vi "FinalProject.vi"() -> ()   [LabVIEW 2016]
uses:
  <vilib>/DAQmx/write.llb/DAQmx Write (Digital Bool 1Line 1Point).vi
  <vilib>/DAQmx/read.llb/DAQmx Read (Digital Bool 1Line 1Point).vi
  <vilib>/DAQmx/create/channels.llb/DAQmx Create Channel (DI-Digital Input).vi
  <vilib>/DAQmx/create/channels.llb/DAQmx Create Channel (DO-Digital Output).vi
  <vilib>/DAQmx/miscellaneous.llb/DAQmx Fill In Error Info.vi
panel:
  out "Pass Test":bool
  out "Overflow Status":bool
  out "Ring Count":i8
  in  "Write File":path
  out "Rejected Plastic":i32
  out "Rejected Metal":i32
  out "Odd Cases":i32
  out "Pass Product":i32
  out "Loading Status":bool
  out "Read File":string
  out "Write File":string
  out "Data Memory":string
  in  "Read File":path
  out "Ring Storage":i8(knob) scale=0.0..5.0
  in  "stop":bool
  out "Stop Button":bool
  out "Top Metal":bool
  out "Top Thing":bool
  out "Top Solenoid":bool
  out "Dropper Thing":bool
  out "Bottom Metal":bool
  out "Assembled":bool
  out "Bottom Solenoid":bool
  out "Bottom Thing":bool
  out "Start Button":bool
  in  "Reject Solenoid":bool
  in  "Belt motor":bool
  in  "Rotary":bool
  in  "Sort Solenoid":bool
  in  "Chain Motor":bool
  # "The overview structure of the program\n\n1. Start every with reading in from the file to retrieve the following data\n\n0: Number of rings in the holder\n1: Ring is loaded\n2: Number of rejeted plastic (Assembled: 0, Metal: 0)\n3: Number of rejected metal (Assembled: 0. Metal: 1)\n4: Number of odd case (Assembled: 1, Metal, 0)\n5: Number of passed product (Assembled: 1, Metal: 1)\n\n2. There are 3 major parts that run simutaneously together\n- Chain motors separates the plastic rings and metals. Exception is the number\nof rings is more than 5, there is nothing to push in (most needed data here)\n- Rotary to load the plastic ring when either there is at least one plastic ring and\nthe Dropper Thing detect empty\n- Assessment process\n\n3. Write in the same memory file in the same order when it started in tab\ndelimeter\n\n4. Repeat the cycle"
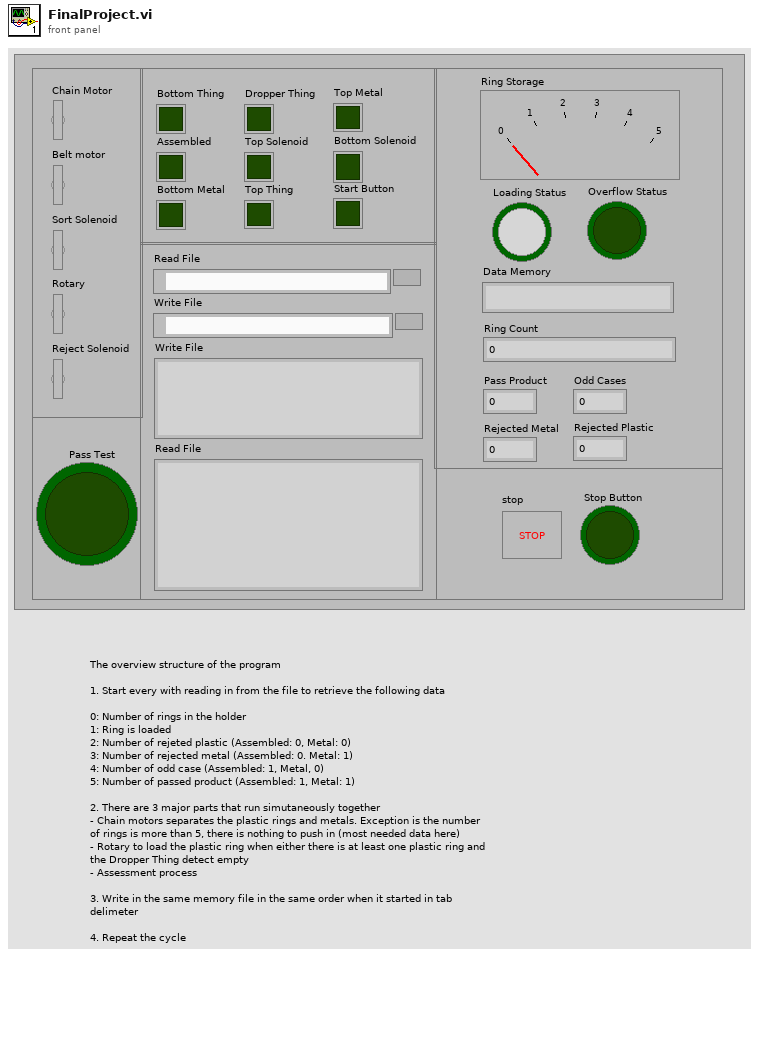
[diagram p1: front panel]
types:
  T1 = enum16{"open", "replace", "create", "open or create", "replace or create", "replace or create with confirmation"}
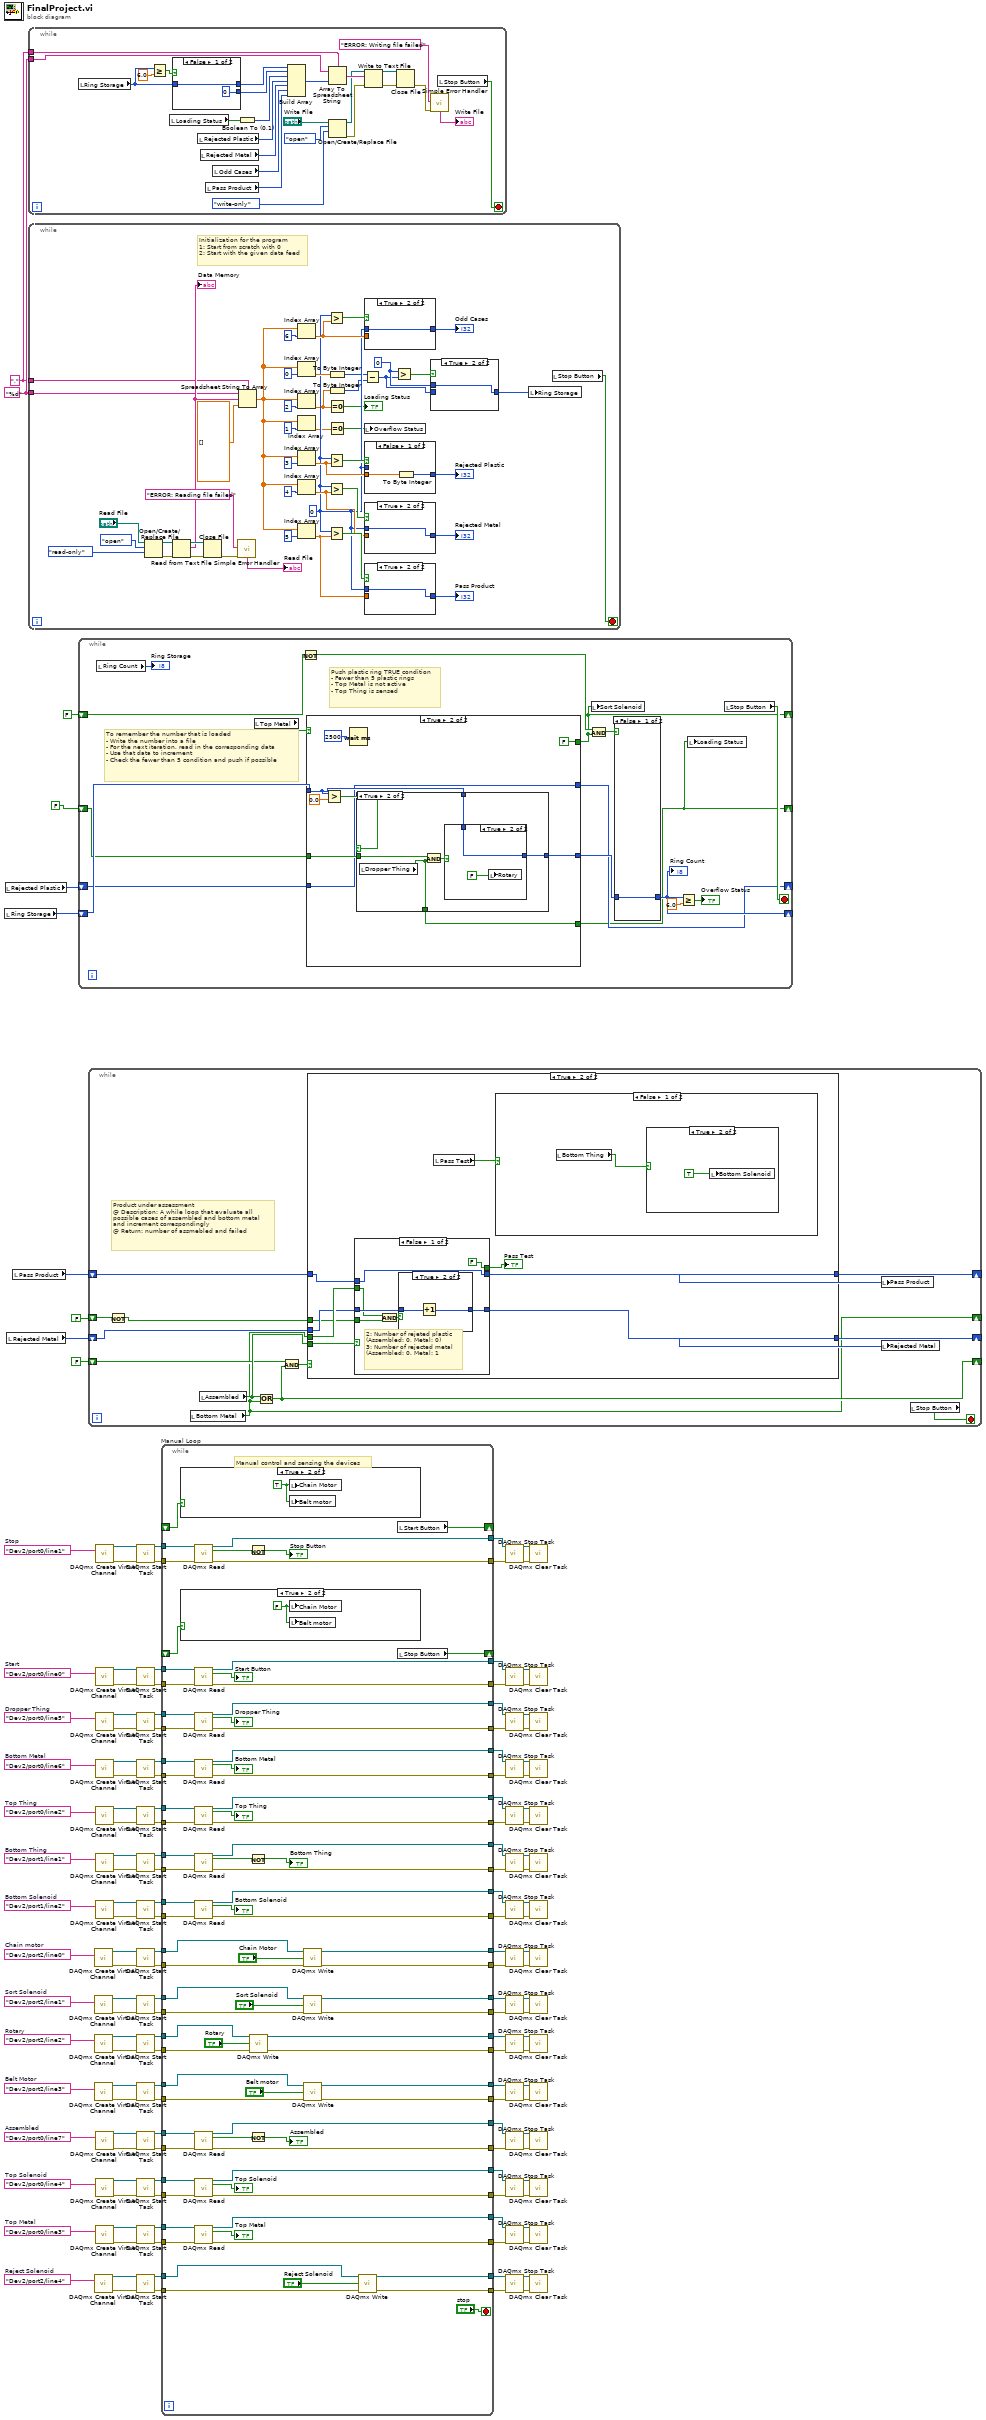
[diagram p0: block diagram]
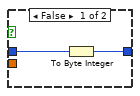
[diagram p2: hidden frame]
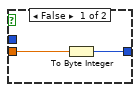
[diagram p3: hidden frame]
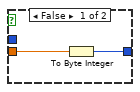
[diagram p4: hidden frame]
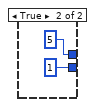
[diagram p7: hidden frame]
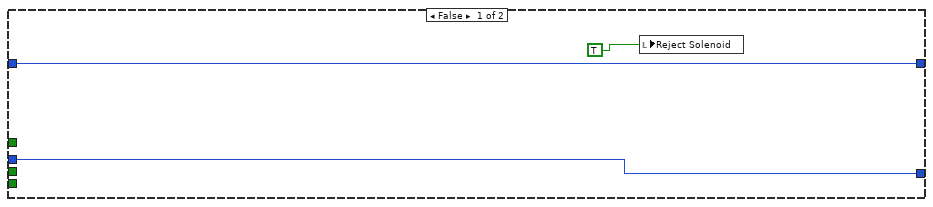
[diagram p8: hidden frame]
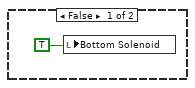
[diagram p9: hidden frame]
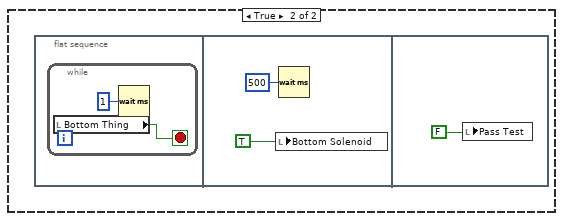
[diagram p10: hidden frame]
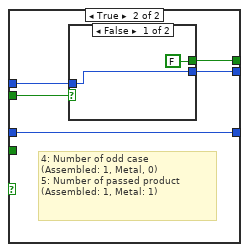
[diagram p12: hidden frame]
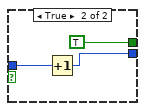
[diagram p13: hidden frame]
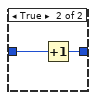
[diagram p14: hidden frame]
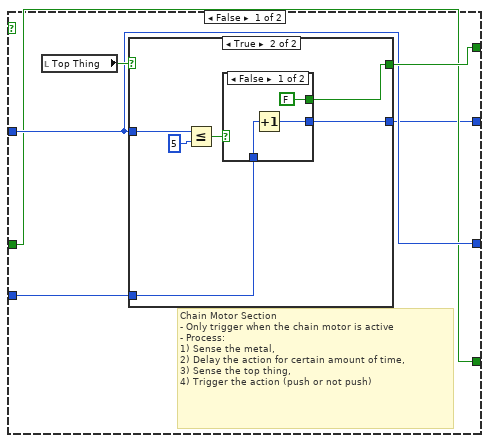
[diagram p15: hidden frame]
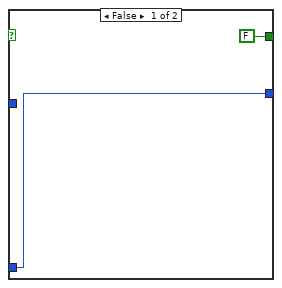
[diagram p16: hidden frame]
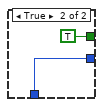
[diagram p17: hidden frame]
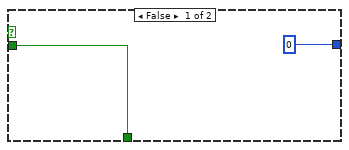
[diagram p18: hidden frame]
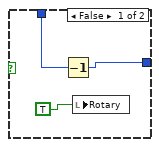
[diagram p19: hidden frame]
diagram:
  w9 = "," ("delimiter (Tab)")
  w10 = "%d" ("format string")
  w105 = tag "Dev2/port1/line2"  # Bottom Solenoid
  w106 = tag "Dev2/port1/line1"  # Bottom Thing
  w111 = tag "Dev2/port0/line7"  # Assembled
  w112 = tag "Dev2/port0/line6"  # Bottom Metal
  w117 = tag "Dev2/port0/line5"  # Dropper Thing
  w118 = tag "Dev2/port0/line4"  # Top Solenoid
  w123 = tag "Dev2/port0/line3"  # Top Metal
  w124 = tag "Dev2/port0/line2"  # Top Thing
  w127 = tag "Dev2/port2/line4"  # Reject Solenoid
  w132 = tag "Dev2/port2/line3"  # Belt Motor
  w133 = tag "Dev2/port2/line2"  # Rotary
  w142 = tag "Dev2/port2/line1"  # Sort Solenoid
  w143 = tag "Dev2/port2/line0"  # Chain motor
  w144 = tag "Dev2/port0/line1"  # Stop
  w145 = tag "Dev2/port0/line0"  # Start
  n1 = local read "Ring Storage"() -> (w8:i8)
  n2 = local read "Rejected Plastic"() -> (w2:i32)
  n3 = local read "Rejected Metal"() -> (w5:i32)
  n4 = local read "Pass Product"() -> (w4:i32)
  n5 = while {
    tunnel: w9 -> [w165]
    tunnel: w10 -> [w164]
    stop <- w157 stop-if-true
    n6 = local read "Ring Storage"() -> (w146:i8)
    n7 = Greater Or Equal?(x=w146, y=6.0) -> (x >= y?=w147:bool)
    n8 = local read "Loading Status"() -> (w155:bool)
    n9 = case shown="False" w147 {
      tunnel: [w172 5] -> w149
      tunnel: [0 1] -> w148
      tunnel: w146 -> [w172 _]
      frame False {
      }
      frame True {
      }
    }
    n10 = local read "Rejected Plastic"() -> (w154:i32)
    n11 = local read "Rejected Metal"() -> (w153:i32)
    n12 = local read "Pass Product"() -> (w151:i32)
    n13 = local read "Odd Cases"() -> (w152:i32)
    n14 = Boolean To (0,1)(Boolean=w155) -> (0, 1=w156:i16)
    n15 = Build Array(w149, w148, w156, w154, w153, w152, w151) -> (w163:i32[])
    n16 = Array To Spreadsheet String(delimiter (Tab)=w165, array=w163, 3:w164) -> (spreadsheet string=w166:string)
    n17 = Open/Create/Replace File(file path (use dialog)="Write File", operation (0:open)=T1."open", access (0:read/write)=enum16{"read/write", "read-only", "write-only"}."write-only") -> (refnum out=w159:refnum<file>, error out=w158:errorcluster)  [unwired: 3 in, 1 out]
    n18 = Write to Text File(file (use dialog)=w159, text=w166, error in=w158) -> (refnum out=w169:refnum<file>, error out=w168:errorcluster)  [unwired: 1 in, 1 out]
    n19 = Close File(refnum=w169, error in=w168) -> (error out=w171:errorcluster)  [unwired: 1 out]
    n20 = call <vilib>:"Simple Error Handler.vi"("error source (\" \")"="ERROR: Writing file failed", "error in (no error)"=w171) -> ("message"=→"Write File":string)  [unwired: 3 in, 4 out]
    n21 = local read "Stop Button"() -> (w157:bool)
  }
  n22 = while {
    tunnel: w10 -> [w192]
    tunnel: w9 -> [w191]
    stop <- w182 stop-if-true
    w205 = 0
    w218 = 0
    # "Initialization for the program\n1: Start from scratch with 0\n2: Start with the given data feed"
    n23 = Open/Create/Replace File(file path (use dialog)="Read File", operation (0:open)=T1."open", access (0:read/write)=enum16{"read/write", "read-only", "write-only"}."read-only") -> (refnum out=w204:refnum<file>, error out=w203:errorcluster)  [unwired: 3 in, 1 out]
    n24 = Read from Text File(file (use dialog)=w204, error in=w203) -> (refnum out=w198:refnum<file>, text=w193:string, error out=w202:errorcluster)  [unwired: 2 in, 1 out]
    "Data Memory" <- w193
    n25 = Close File(refnum=w198, error in=w202) -> (error out=w196:errorcluster)  [unwired: 1 out]
    n26 = call <vilib>:"Simple Error Handler.vi"("error source (\" \")"="ERROR: Reading file failed", "error in (no error)"=w196) -> ("message"=→"Read File":string)  [unwired: 3 in, 4 out]
    n27 = Spreadsheet String To Array(delimiter (Tab)=w191, format string=w192, spreadsheet string=w193, array type (2D Dbl)=dbl[] []) -> (array=w179:dbl[])
    n28 = Index Array(array=w179, index=6) -> (element=w206:dbl)
    n29 = Index Array(array=w179, index=0 ("index (vol)")) -> (element=w222:dbl)
    n30 = Index Array(array=w179, index=2) -> (element=w186:dbl)
    n31 = Index Array(array=w179, index=1 ("index (vol)")) -> (element=w176:dbl)
    n32 = Index Array(array=w179, index=3) -> (element=w209:dbl)
    n33 = Index Array(array=w179, index=4) -> (element=w208:dbl)
    n34 = Index Array(array=w179, index=5) -> (element=w207:dbl)
    n35 = Greater?(x=w205, y=w206) -> (0:w210:bool)
    n36 = Greater?(x=w205, y=w209) -> (0:w213:bool)
    n37 = Greater?(x=w205, y=w208) -> (0:w212:bool)
    n38 = Greater?(x=w205, y=w207) -> (0:w211:bool)
    n39 = To Byte Integer(number=w222) -> (8bit integer=w185:i8)
    n40 = To Byte Integer(number=w186) -> (8bit integer=w184:i8)
    n41 = Equal To 0?(x=w186) -> (x = 0?=→"Loading Status":bool)
    n42 = Equal To 0?(x=w176) -> (x = 0?=w177:bool)
    n43 = Subtract(x=w185, y=w184) -> (x-y=w183:i8)
    n44 = case shown="True" w210 {
      tunnel: [w224 w225] -> w187
      tunnel: w206 -> [_ _]
      tunnel: w205 -> [w223 w225]
      frame False {
        n45 = To Byte Integer(number=w223) -> (8bit integer=w224:i8)
      }
      frame True {
      }
    }
    "Odd Cases" <- w187
    n46 = local write "Overflow Status"(w177) -> ()
    n47 = case shown="False" w213 {
      tunnel: [w232 w234] -> w190
      tunnel: w205 -> [_ w234]
      tunnel: w209 -> [w233 _]
      frame False {
        n48 = To Byte Integer(number=w233) -> (8bit integer=w232:i8)
      }
      frame True {
      }
    }
    "Rejected Plastic" <- w190
    n49 = case shown="True" w212 {
      tunnel: [w229 w231] -> w189
      tunnel: w205 -> [_ w231]
      tunnel: w208 -> [w230 _]
      frame False {
        n50 = To Byte Integer(number=w230) -> (8bit integer=w229:i8)
      }
      frame True {
      }
    }
    "Rejected Metal" <- w189
    n51 = case shown="True" w211 {
      tunnel: [w226 w228] -> w188
      tunnel: w205 -> [_ w228]
      tunnel: w207 -> [w227 _]
      frame False {
        n52 = To Byte Integer(number=w227) -> (8bit integer=w226:i8)
      }
      frame True {
      }
    }
    "Pass Product" <- w188
    n53 = Greater?(x=w218, y=w183) -> (0:w219:bool)
    n54 = case shown="True" w219 {
      tunnel: [w235 w236] -> w181
      tunnel: w218 -> [_ w236]
      tunnel: w183 -> [w235 _]
      frame False {
      }
      frame True {
      }
    }
    n55 = local write "Ring Storage"(w181) -> ()
    n56 = local read "Stop Button"() -> (w182:bool)
  }
  n57 = while {
    shift-right: [w242] -> _
    shift-left: w8 -> [w250]
    shift-right: [w246] -> _
    shift-left: FALSE -> [w247]
    shift-right: [w237] -> _
    shift-left: FALSE -> [w241]
    shift-right: [w238] -> _
    shift-left: w2 -> [w239]
    stop <- w251 stop-if-true
    # "Push plastic ring TRUE condition\n- Fewer than 5 plastic rings\n- Top Metal is not active\n- Top Thing is sensed"
    # "To remember the number that is loaded\n- Write the number into a file\n- For the next iteration, read in the corresponding data\n- Use that data to increment\n- Check the fewer than 5 condition and push if possible"
    n58 = local read "Ring Count"() -> (→"Ring Storage":i8)
    n59 = local read "Top Metal"() -> (w252:bool)
    n60 = Not(x=w247) -> (.not. x?=w248:bool)
    n61 = case shown="True" w252 {
      tunnel: [w260 FALSE] -> w246
      tunnel: w250 -> [w259 w277]
      tunnel: w241 -> [w258 w279]
      tunnel: [w258 w278] -> w237
      tunnel: [w259 w276] -> w240
      tunnel: w239 -> [w257 w275]
      tunnel: [w256 w275] -> w238
      frame False {
        # "Chain Motor Section\n- Only trigger when the chain motor is active\n- Process: \n1) Sense the metal, \n2) Delay the action for certain amount of time, \n3) Sense the top thing,\n4) Trigger the action (push or not push)"
        n62 = local read "Top Thing"() -> (w261:bool)
        n63 = case shown="True" w261 {
          tunnel: [FALSE w267] -> w260
          tunnel: w259 -> [_ w266]
          tunnel: w257 -> [w262 w265]
          tunnel: [w262 w264] -> w256
          frame False {
          }
          frame True {
            n64 = Less Or Equal?(x=w266, y=i8 5) -> (x <= y?=w268:bool)
            n65 = case shown="False" w268 {
              tunnel: [FALSE TRUE] -> w267
              tunnel: w265 -> [w271 w273]
              tunnel: [w270 w273] -> w264
              frame False {
                n66 = Increment(x=w271) -> (x+1=w270:i32)
              }
              frame True {
              }
            }
          }
        }
      }
      frame True {
        n67 = Greater?(x=w277, y=0.0) -> (0:w280:bool)
        n68 = Wait (ms)(milliseconds to wait=u32 2500 ("millisecond timer value")) -> ()  [unwired: 1 out]
        n69 = case shown="True" w280 {
          tunnel: w279 -> [w284 w289]
          tunnel: [w284 w288] -> w278
          tunnel: w277 -> [_ w287]
          tunnel: [0 w286] -> w276
          frame False {
          }
          frame True {
            n70 = local read "Dropper Thing"() -> (w288:bool)
            n71 = And(x=w289, y=w288) -> (x .and. y?=w290:bool)
            n72 = case shown="True" w290 {
              tunnel: w287 -> [w292 w295]
              tunnel: [w293 w295] -> w286
              frame False {
                n73 = Decrement(x=w292) -> (x-1=w293:i32)
                n74 = local write "Rotary"(TRUE) -> ()
              }
              frame True {
                n75 = local write "Rotary"(FALSE) -> ()
              }
            }
          }
        }
      }
    }
    n76 = And(x=w248, y=w246) -> (x .and. y?=w249:bool)
    n77 = local write "Sort Solenoid"(w246) -> ()
    n78 = case shown="False" w249 {
      tunnel: [w253 w254] -> w242
      tunnel: w240 -> [w253 w255]
      frame False {
      }
      frame True {
        n79 = Increment(x=w255) -> (x+1=w254:i32)
      }
    }
    "Ring Count" <- w242
    n80 = Greater Or Equal?(x=w242, y=6.0) -> (x >= y?=→"Overflow Status":bool)
    n81 = local write "Loading Status"(w237) -> ()
    n82 = local read "Stop Button"() -> (w251:bool)
  }
  n83 = while {
    shift-right: [w303] -> _
    shift-left: FALSE -> [w305]
    shift-right: [w300] -> _
    shift-left: w5 -> [w302]
    shift-right: [w299] -> _
    shift-left: w4 -> [w301]
    shift-right: [w296] -> _
    shift-left: FALSE -> [w298]
    stop <- w307 stop-if-true
    # "Product under assessment\n@ Description: A while loop that evaluate all \npossible cases of assembled and bottom metal\nand increment correspondingly\n@ Return: number of assmebled and failed"
    n84 = Not(x=w298) -> (.not. x?=w297:bool)
    n85 = local read "Bottom Metal"() -> (w296:bool)
    n86 = local read "Assembled"() -> (w306:bool)
    n87 = Or(x=w306, y=w296) -> (x .or. y?=w303:bool)
    n88 = And(x=w305, y=w303) -> (x .and. y?=w304:bool)
    n89 = case shown="True" w304 {
      tunnel: w306 -> [_ w316]
      tunnel: w296 -> [_ w317]
      tunnel: w302 -> [w310 w315]
      tunnel: w301 -> [w309 w319]
      tunnel: [w310 w314] -> w300
      tunnel: [w309 w318] -> w299
      tunnel: w297 -> [_ w311]
      frame False {
        n90 = local write "Reject Solenoid"(TRUE) -> ()
      }
      frame True {
        n91 = case shown="False" w316 {
          tunnel: w319 -> [w334 w339]
          tunnel: [w334 w342] -> w318
          tunnel: w317 -> [w329 w341]
          tunnel: w315 -> [w333 w340]
          tunnel: [w332 w340] -> w314
          tunnel: [FALSE w338] -> w312
          tunnel: w311 -> [w328 _]
          frame False {
            # "2: Number of rejeted plastic\n(Assembled: 0, Metal: 0)\n3: Number of rejected metal\n(Assembled: 0. Metal: 1"
            n92 = And(x=w329, y=w328) -> (x .and. y?=w330:bool)
            n93 = case shown="True" w330 {
              tunnel: w333 -> [w335 w337]
              tunnel: [w335 w336] -> w332
              frame False {
              }
              frame True {
                n94 = Increment(x=w337) -> (x+1=w336:i32)
              }
            }
          }
          frame True {
            # "4: Number of odd case\n(Assembled: 1, Metal, 0)\n5: Number of passed product\n(Assembled: 1, Metal: 1)"
            n95 = case shown="False" w341 {
              tunnel: w339 -> [w344 w346]
              tunnel: [w344 w347] -> w342
              tunnel: [FALSE TRUE] -> w338
              frame False {
              }
              frame True {
                n96 = Increment(x=w346) -> (x+1=w347:i32)
              }
            }
          }
        }
        "Pass Test" <- w312
        n97 = local read "Pass Test"() -> (w313:bool)
        n98 = case shown="False" w313 {
          frame False {
            n99 = local read "Bottom Thing"() -> (w320:bool)
            n100 = case shown="True" w320 {
              frame False {
                n101 = local write "Bottom Solenoid"(TRUE) -> ()
              }
              frame True {
                n102 = local write "Bottom Solenoid"(TRUE) -> ()
              }
            }
          }
          frame True {
            n103 = flat-sequence {
              frame #0 {
                n104 = while {
                  stop <- w323 stop-if-true
                  n105 = local read "Bottom Thing"() -> (w323:bool)
                  n106 = Wait (ms)(milliseconds to wait=u32 1) -> ()  [unwired: 1 out]
                }
              }
              frame #1 {
                n107 = local write "Bottom Solenoid"(TRUE) -> ()
                n108 = Wait (ms)(milliseconds to wait=u32 500) -> ()  [unwired: 1 out]
              }
              frame #2 {
                n109 = local write "Pass Test"(FALSE) -> ()
              }
            }
          }
        }
      }
    }
    n110 = local write "Pass Product"(w299) -> ()
    n111 = local write "Rejected Metal"(w300) -> ()
    n112 = local read "Stop Button"() -> (w307:bool)
  }
  n113 = call-poly <vilib>:"DAQmx Create Virtual Channel.vi"("lines"=w143) -> ("task out"=w137:refnum<k21>, "error out"=w136:errorcluster)  [unwired: 13 in]
  n114 = call-poly <vilib>:"DAQmx Create Virtual Channel.vi"("lines"=w142) -> ("task out"=w135:refnum<k21>, "error out"=w134:errorcluster)  [unwired: 13 in]
  n115 = call-poly <vilib>:"DAQmx Create Virtual Channel.vi"("lines"=w133) -> ("task out"=w131:refnum<k21>, "error out"=w130:errorcluster)  [unwired: 13 in]
  n116 = call-poly <vilib>:"DAQmx Create Virtual Channel.vi"("lines"=w132) -> ("task out"=w129:refnum<k21>, "error out"=w128:errorcluster)  [unwired: 13 in]
  n117 = call-poly <vilib>:"DAQmx Create Virtual Channel.vi"("lines"=w127) -> ("task out"=w126:refnum<k21>, "error out"=w125:errorcluster)  [unwired: 13 in]
  n118 = call-poly <vilib>:"DAQmx Create Virtual Channel.vi"("lines"=w144) -> ("task out"=w139:refnum<k21>, "error out"=w138:errorcluster)  [unwired: 13 in]
  n119 = call-poly <vilib>:"DAQmx Create Virtual Channel.vi"("lines"=w145) -> ("task out"=w140:refnum<k21>, "error out"=w141:errorcluster)  [unwired: 13 in]
  n120 = call-poly <vilib>:"DAQmx Create Virtual Channel.vi"("lines"=w117) -> ("task out"=w114:refnum<k21>, "error out"=w113:errorcluster)  [unwired: 13 in]
  n121 = call-poly <vilib>:"DAQmx Create Virtual Channel.vi"("lines"=w112) -> ("task out"=w109:refnum<k21>, "error out"=w110:errorcluster)  [unwired: 13 in]
  n122 = call-poly <vilib>:"DAQmx Create Virtual Channel.vi"("lines"=w124) -> ("task out"=w121:refnum<k21>, "error out"=w122:errorcluster)  [unwired: 13 in]
  n123 = call-poly <vilib>:"DAQmx Create Virtual Channel.vi"("lines"=w106) -> ("task out"=w103:refnum<k21>, "error out"=w104:errorcluster)  [unwired: 13 in]
  n124 = call-poly <vilib>:"DAQmx Create Virtual Channel.vi"("lines"=w105) -> ("task out"=w102:refnum<k21>, "error out"=w101:errorcluster)  [unwired: 13 in]
  n125 = call-poly <vilib>:"DAQmx Create Virtual Channel.vi"("lines"=w111) -> ("task out"=w108:refnum<k21>, "error out"=w107:errorcluster)  [unwired: 13 in]
  n126 = call-poly <vilib>:"DAQmx Create Virtual Channel.vi"("lines"=w118) -> ("task out"=w115:refnum<k21>, "error out"=w116:errorcluster)  [unwired: 13 in]
  n127 = call-poly <vilib>:"DAQmx Create Virtual Channel.vi"("lines"=w123) -> ("task out"=w120:refnum<k21>, "error out"=w119:errorcluster)  [unwired: 13 in]
  n128 = call <vilib>:"DAQmx Start Task.vi"("task/channels in"=w139, "error in"=w138) -> ("task out"=w98:refnum<k21>, "error out"=w97:errorcluster)  [unwired: 12 in]
  n129 = call <vilib>:"DAQmx Start Task.vi"("task/channels in"=w140, "error in"=w141) -> ("task out"=w100:refnum<k21>, "error out"=w99:errorcluster)  [unwired: 12 in]
  n130 = call <vilib>:"DAQmx Start Task.vi"("task/channels in"=w114, "error in"=w113) -> ("task out"=w37:refnum<k21>, "error out"=w38:errorcluster)  [unwired: 12 in]
  n131 = call <vilib>:"DAQmx Start Task.vi"("task/channels in"=w109, "error in"=w110) -> ("task out"=w40:refnum<k21>, "error out"=w39:errorcluster)  [unwired: 12 in]
  n132 = call <vilib>:"DAQmx Start Task.vi"("task/channels in"=w121, "error in"=w122) -> ("task out"=w88:refnum<k21>, "error out"=w87:errorcluster)  [unwired: 12 in]
  n133 = call <vilib>:"DAQmx Start Task.vi"("task/channels in"=w103, "error in"=w104) -> ("task out"=w54:refnum<k21>, "error out"=w53:errorcluster)  [unwired: 12 in]
  n134 = call <vilib>:"DAQmx Start Task.vi"("task/channels in"=w102, "error in"=w101) -> ("task out"=w50:refnum<k21>, "error out"=w49:errorcluster)  [unwired: 12 in]
  n135 = call <vilib>:"DAQmx Start Task.vi"("task/channels in"=w137, "error in"=w136) -> ("task out"=w30:refnum<k21>, "error out"=w29:errorcluster)  [unwired: 12 in]
  n136 = call <vilib>:"DAQmx Start Task.vi"("task/channels in"=w135, "error in"=w134) -> ("task out"=w28:refnum<k21>, "error out"=w27:errorcluster)  [unwired: 12 in]
  n137 = call <vilib>:"DAQmx Start Task.vi"("task/channels in"=w131, "error in"=w130) -> ("task out"=w12:refnum<k21>, "error out"=w11:errorcluster)  [unwired: 12 in]
  n138 = call <vilib>:"DAQmx Start Task.vi"("task/channels in"=w129, "error in"=w128) -> ("task out"=w16:refnum<k21>, "error out"=w15:errorcluster)  [unwired: 12 in]
  n139 = call <vilib>:"DAQmx Start Task.vi"("task/channels in"=w108, "error in"=w107) -> ("task out"=w46:refnum<k21>, "error out"=w45:errorcluster)  [unwired: 12 in]
  n140 = call <vilib>:"DAQmx Start Task.vi"("task/channels in"=w115, "error in"=w116) -> ("task out"=w34:refnum<k21>, "error out"=w33:errorcluster)  [unwired: 12 in]
  n141 = call <vilib>:"DAQmx Start Task.vi"("task/channels in"=w120, "error in"=w119) -> ("task out"=w80:refnum<k21>, "error out"=w79:errorcluster)  [unwired: 12 in]
  n142 = call <vilib>:"DAQmx Start Task.vi"("task/channels in"=w126, "error in"=w125) -> ("task out"=w22:refnum<k21>, "error out"=w21:errorcluster)  [unwired: 12 in]
  n143 = while "Manual Loop" {
    tunnel: w100 -> [w429]
    tunnel: w99 -> [w428]
    tunnel: w98 -> [w425]
    tunnel: w97 -> [w424]
    tunnel: [w423] -> w94
    tunnel: [w422] -> w93
    tunnel: [w421] -> w90
    tunnel: [w420] -> w89
    tunnel: w88 -> [w419]
    tunnel: w87 -> [w418]
    tunnel: [w417] -> w84
    tunnel: [w416] -> w83
    tunnel: w80 -> [w415]
    tunnel: w79 -> [w414]
    tunnel: [w413] -> w78
    tunnel: [w412] -> w77
    tunnel: w54 -> [w411]
    tunnel: w53 -> [w410]
    tunnel: [w409] -> w52
    tunnel: [w408] -> w51
    tunnel: w50 -> [w407]
    tunnel: w49 -> [w406]
    tunnel: [w405] -> w48
    tunnel: [w404] -> w47
    tunnel: w46 -> [w402]
    tunnel: w45 -> [w401]
    tunnel: [w400] -> w44
    tunnel: [w399] -> w43
    tunnel: [w398] -> w42
    tunnel: [w397] -> w41
    tunnel: w40 -> [w396]
    tunnel: w39 -> [w395]
    tunnel: w38 -> [w394]
    tunnel: w37 -> [w393]
    tunnel: [w392] -> w36
    tunnel: [w391] -> w35
    tunnel: w34 -> [w390]
    tunnel: w33 -> [w389]
    tunnel: [w388] -> w32
    tunnel: [w387] -> w31
    tunnel: w30 -> [w386]
    tunnel: w29 -> [w385]
    tunnel: w28 -> [w384]
    tunnel: w27 -> [w383]
    tunnel: [w382] -> w26
    tunnel: [w381] -> w25
    tunnel: [w380] -> w24
    tunnel: [w379] -> w23
    tunnel: w22 -> [w378]
    tunnel: w21 -> [w377]
    tunnel: [w376] -> w20
    tunnel: [w375] -> w19
    tunnel: [w374] -> w18
    tunnel: [w373] -> w17
    tunnel: w16 -> [w372]
    tunnel: w15 -> [w371]
    tunnel: [w370] -> w14
    tunnel: [w369] -> w13
    tunnel: w12 -> [w368]
    tunnel: w11 -> [w367]
    shift-right: [w362] -> _
    shift-left: _ -> [w357]
    shift-right: [w361] -> _
    shift-left: _ -> [w358]
    stop <- "stop" stop-if-true
    # "Manual control and sensing the devices"
    n144 = case shown="True" w357 {
      frame False {
      }
      frame True {
        w431 = TRUE
        n145 = local write "Chain Motor"(w431) -> ()
        n146 = local write "Belt motor"(w431) -> ()
      }
    }
    n147 = case shown="True" w358 {
      frame False {
      }
      frame True {
        w432 = FALSE
        n148 = local write "Chain Motor"(w432) -> ()
        n149 = local write "Belt motor"(w432) -> ()
      }
    }
    n150 = call-poly <vilib>:"DAQmx Read.vi"("task/channels in"=w425, "error in"=w424) -> ("task out"=w423:refnum<k21>, "data"=w427:bool, "error out"=w422:errorcluster)  [unwired: 11 in]
    n151 = call-poly <vilib>:"DAQmx Read.vi"("task/channels in"=w429, "error in"=w428) -> ("task out"=w421:refnum<k21>, "data"=→"Start Button":bool, "error out"=w420:errorcluster)  [unwired: 11 in]
    n152 = call-poly <vilib>:"DAQmx Read.vi"("task/channels in"=w393, "error in"=w394) -> ("task out"=w392:refnum<k21>, "data"=→"Dropper Thing":bool, "error out"=w391:errorcluster)  [unwired: 11 in]
    n153 = call-poly <vilib>:"DAQmx Read.vi"("task/channels in"=w396, "error in"=w395) -> ("task out"=w398:refnum<k21>, "data"=→"Bottom Metal":bool, "error out"=w397:errorcluster)  [unwired: 11 in]
    n154 = call-poly <vilib>:"DAQmx Read.vi"("task/channels in"=w419, "error in"=w418) -> ("task out"=w416:refnum<k21>, "data"=→"Top Thing":bool, "error out"=w417:errorcluster)  [unwired: 11 in]
    n155 = call-poly <vilib>:"DAQmx Read.vi"("task/channels in"=w411, "error in"=w410) -> ("task out"=w409:refnum<k21>, "data"=w348:bool, "error out"=w408:errorcluster)  [unwired: 11 in]
    n156 = call-poly <vilib>:"DAQmx Read.vi"("task/channels in"=w407, "error in"=w406) -> ("task out"=w405:refnum<k21>, "data"=→"Bottom Solenoid":bool, "error out"=w404:errorcluster)  [unwired: 11 in]
    n157 = call-poly <vilib>:"DAQmx Read.vi"("task/channels in"=w402, "error in"=w401) -> ("task out"=w400:refnum<k21>, "data"=w350:bool, "error out"=w399:errorcluster)  [unwired: 11 in]
    n158 = call-poly <vilib>:"DAQmx Read.vi"("task/channels in"=w390, "error in"=w389) -> ("task out"=w388:refnum<k21>, "data"=→"Top Solenoid":bool, "error out"=w387:errorcluster)  [unwired: 11 in]
    n159 = call-poly <vilib>:"DAQmx Read.vi"("task/channels in"=w415, "error in"=w414) -> ("task out"=w413:refnum<k21>, "data"=→"Top Metal":bool, "error out"=w412:errorcluster)  [unwired: 11 in]
    n160 = Not(x=w427) -> (.not. x?=→"Stop Button":bool)
    n161 = Not(x=w348) -> (.not. x?=→"Bottom Thing":bool)
    n162 = call-poly <vilib>:"DAQmx Write.vi"("task/channels in"=w368, "data"="Rotary", "error in"=w367) -> ("task out"=w369:refnum<k21>, "error out"=w370:errorcluster)  [unwired: 10 in, 1 out]
    n163 = Not(x=w350) -> (.not. x?=→"Assembled":bool)
    n164 = call-poly <vilib>:"DAQmx Write.vi"("task/channels in"=w386, "data"="Chain Motor", "error in"=w385) -> ("task out"=w382:refnum<k21>, "error out"=w381:errorcluster)  [unwired: 10 in, 1 out]
    n165 = call-poly <vilib>:"DAQmx Write.vi"("task/channels in"=w384, "data"="Sort Solenoid", "error in"=w383) -> ("task out"=w380:refnum<k21>, "error out"=w379:errorcluster)  [unwired: 10 in, 1 out]
    n166 = call-poly <vilib>:"DAQmx Write.vi"("task/channels in"=w372, "data"="Belt motor", "error in"=w371) -> ("task out"=w374:refnum<k21>, "error out"=w373:errorcluster)  [unwired: 10 in, 1 out]
    n167 = call-poly <vilib>:"DAQmx Write.vi"("task/channels in"=w378, "data"="Reject Solenoid", "error in"=w377) -> ("task out"=w376:refnum<k21>, "error out"=w375:errorcluster)  [unwired: 10 in, 1 out]
    n168 = local read "Start Button"() -> (w362:bool)
    n169 = local read "Stop Button"() -> (w361:bool)
  }
  n170 = call <vilib>:"DAQmx Stop Task.vi"("task/channels in"=w94, "error in"=w93) -> ("task out"=w95:refnum<k21>, "error out"=w96:errorcluster)  [unwired: 12 in]
  n171 = call <vilib>:"DAQmx Stop Task.vi"("task/channels in"=w90, "error in"=w89) -> ("task out"=w91:refnum<k21>, "error out"=w92:errorcluster)  [unwired: 12 in]
  n172 = call <vilib>:"DAQmx Stop Task.vi"("task/channels in"=w36, "error in"=w35) -> ("task out"=w65:refnum<k21>, "error out"=w66:errorcluster)  [unwired: 12 in]
  n173 = call <vilib>:"DAQmx Stop Task.vi"("task/channels in"=w42, "error in"=w41) -> ("task out"=w63:refnum<k21>, "error out"=w64:errorcluster)  [unwired: 12 in]
  n174 = call <vilib>:"DAQmx Stop Task.vi"("task/channels in"=w83, "error in"=w84) -> ("task out"=w85:refnum<k21>, "error out"=w86:errorcluster)  [unwired: 12 in]
  n175 = call <vilib>:"DAQmx Stop Task.vi"("task/channels in"=w52, "error in"=w51) -> ("task out"=w75:refnum<k21>, "error out"=w76:errorcluster)  [unwired: 12 in]
  n176 = call <vilib>:"DAQmx Stop Task.vi"("task/channels in"=w48, "error in"=w47) -> ("task out"=w73:refnum<k21>, "error out"=w74:errorcluster)  [unwired: 12 in]
  n177 = call <vilib>:"DAQmx Stop Task.vi"("task/channels in"=w26, "error in"=w25) -> ("task out"=w71:refnum<k21>, "error out"=w72:errorcluster)  [unwired: 12 in]
  n178 = call <vilib>:"DAQmx Stop Task.vi"("task/channels in"=w24, "error in"=w23) -> ("task out"=w69:refnum<k21>, "error out"=w70:errorcluster)  [unwired: 12 in]
  n179 = call <vilib>:"DAQmx Stop Task.vi"("task/channels in"=w13, "error in"=w14) -> ("task out"=w59:refnum<k21>, "error out"=w60:errorcluster)  [unwired: 12 in]
  n180 = call <vilib>:"DAQmx Stop Task.vi"("task/channels in"=w18, "error in"=w17) -> ("task out"=w57:refnum<k21>, "error out"=w58:errorcluster)  [unwired: 12 in]
  n181 = call <vilib>:"DAQmx Stop Task.vi"("task/channels in"=w44, "error in"=w43) -> ("task out"=w61:refnum<k21>, "error out"=w62:errorcluster)  [unwired: 12 in]
  n182 = call <vilib>:"DAQmx Stop Task.vi"("task/channels in"=w32, "error in"=w31) -> ("task out"=w67:refnum<k21>, "error out"=w68:errorcluster)  [unwired: 12 in]
  n183 = call <vilib>:"DAQmx Stop Task.vi"("task/channels in"=w78, "error in"=w77) -> ("task out"=w81:refnum<k21>, "error out"=w82:errorcluster)  [unwired: 12 in]
  n184 = call <vilib>:"DAQmx Stop Task.vi"("task/channels in"=w20, "error in"=w19) -> ("task out"=w55:refnum<k21>, "error out"=w56:errorcluster)  [unwired: 12 in]
  n185 = call <vilib>:"DAQmx Clear Task.vi"("task in"=w95, "error in"=w96) -> ()  [unwired: 13 in, 1 out]
  n186 = call <vilib>:"DAQmx Clear Task.vi"("task in"=w91, "error in"=w92) -> ()  [unwired: 13 in, 1 out]
  n187 = call <vilib>:"DAQmx Clear Task.vi"("task in"=w65, "error in"=w66) -> ()  [unwired: 13 in, 1 out]
  n188 = call <vilib>:"DAQmx Clear Task.vi"("task in"=w63, "error in"=w64) -> ()  [unwired: 13 in, 1 out]
  n189 = call <vilib>:"DAQmx Clear Task.vi"("task in"=w85, "error in"=w86) -> ()  [unwired: 13 in, 1 out]
  n190 = call <vilib>:"DAQmx Clear Task.vi"("task in"=w75, "error in"=w76) -> ()  [unwired: 13 in, 1 out]
  n191 = call <vilib>:"DAQmx Clear Task.vi"("task in"=w73, "error in"=w74) -> ()  [unwired: 13 in, 1 out]
  n192 = call <vilib>:"DAQmx Clear Task.vi"("task in"=w71, "error in"=w72) -> ()  [unwired: 13 in, 1 out]
  n193 = call <vilib>:"DAQmx Clear Task.vi"("task in"=w69, "error in"=w70) -> ()  [unwired: 13 in, 1 out]
  n194 = call <vilib>:"DAQmx Clear Task.vi"("task in"=w59, "error in"=w60) -> ()  [unwired: 13 in, 1 out]
  n195 = call <vilib>:"DAQmx Clear Task.vi"("task in"=w57, "error in"=w58) -> ()  [unwired: 13 in, 1 out]
  n196 = call <vilib>:"DAQmx Clear Task.vi"("task in"=w61, "error in"=w62) -> ()  [unwired: 13 in, 1 out]
  n197 = call <vilib>:"DAQmx Clear Task.vi"("task in"=w67, "error in"=w68) -> ()  [unwired: 13 in, 1 out]
  n198 = call <vilib>:"DAQmx Clear Task.vi"("task in"=w81, "error in"=w82) -> ()  [unwired: 13 in, 1 out]
  n199 = call <vilib>:"DAQmx Clear Task.vi"("task in"=w55, "error in"=w56) -> ()  [unwired: 13 in, 1 out]
